vi "AnalysisTools.vi"(7 "Cali.Ref(Caller)":refnum<vi>) -> ()   [LabVIEW 2013]
uses:
  ProcessMethods/Binning/BinType.ctl
  <vilib>/Utility/miscctls.llb/LVRowAndColumnUnsignedTypeDef.ctl
  Files/Signal_Segment.ctl
  ControlDef/ProcessingMode.ctl
  <vilib>/Analysis/6fits.llb/General Linear Fit Algorithm.ctl
  <vilib>/Analysis/6fits.llb/Curve Fitting Criteria.ctl
  UI/Autoscale_Y_Multiple.vi
  ProcessMethods/Binning/SpectraBinning.vi
  ProcessMethods/MassResolutionCalc/FindMassResolution_Multiple.vi
  <vilib>/regexp/Match Regular Expression.xnode
  <vilib>/Analysis/NI_AALPro.lvlib
  <vilib>/Analysis/NI_AAL_SigProc.lvlib
  <vilib>/ptbypt/NI_PtbyPt.lvlib
panel:
  in  "Resolution":bool
  in  "Binning":bool
  in  "BinType":T1
  in  "BinWidth":dbl=1.0 min=0.001 max=32768.0 step=0.001 format="%.3f"
  in  "X++":bool
  in  "X--":bool
  in  "Fullscale X":bool
  in  "Fullscale Y":bool
  in  "Y--":bool
  in  "Y++":bool
  in  "Reload":bool
  in  "Path":path
  out "Spectrum":cluster{dbl[], "Amplitudes":dbl[]}[](graph)
  in  "Calc Calibration":bool
  in  "m/z":dbl
  in  "time":dbl
  in  "Add to":bool
  out "Original m/z":dbl
  in  "Tab Control":T2(tab)
  in  "Calibration Table":dbl[][](array[numeric]) caption="raw m/z"
  in  "Quit":bool
  in  "Export_GraphData":bool
  in  "ApplyToFile":bool
  out "M/z curve fitting":cluster{"Y":dbl[], "Y":dbl[]}[](graph)
  in  "Calibration Coefficients":dbl[](array[numeric]) format="%.5f"
  out "R^2":dbl
  in  "Apply":bool
  in  "mzML Export":bool
  in  "ApplyToMainProgram":bool
  in  "AddSelection":bool
  in  "ExportPCA":bool
  in  "Multicolumn Listbox":i32[](listbox)
  in  "Search":bool
  in  "threshold":dbl format="%#_5p"
  in  "width":i32=3 min=3
  out "# found":i32
  in  "LoadMultiple...":bool
  in  "Reset":bool
  in  "ExportTable":bool
  in  "CopyPeakAreas":bool
  in  "CalcPeakAreas":bool
  in  "Selected Peak list":i32[](listbox)=[2]
  in  "Decode_regexp":string="Br2-Tyr_([-+]?[0-9]*[,\\.]?[0-9]+([eE][-+]?[0-9]+)?)%_([-+]?[0-9]*[,\\.]?[0-9]+([eE][-+]?[0-9]+)?)uJ_([-+]?[0-9]*[,\\.]?[0-9]+([eE][-+]?[0-9]+)?)us_([-+]?[0-9]*[,\\.]?[0-9]+([eE][-+]?[0-9]+)?).txt"
  in  "Decode_Filename?":bool
  in  "Accumulate":bool
  out "Accumulated Data":dbl[][](array[numeric])
  in  "Export+Proc":bool
  out "selected submatch":string
  in  "Submatch Selector":i32
  out "Referance Mass":string[][](table)=[["Compound", "", "mass", ""], ["Sexithiophone", "6T", "493.98", "s"], ["", "4T", "330.00", "s"], ["", "8T", "657.96", "w"], ["NPM", "M+", "297", "s"], ["", "", "217", "w"], ["CHCA", "M+", "189.04", "s"], ["DHB", "M+", "154.03", "s"], ["Rifampcin", "", "", ""], ["Tantalum", "", "", ""], ["Cu", "63", "", ""], ["", "65", "", ""], ["Mo", "", "", ""]]
  # "raw m/z"
  # "time"
  # "cali. m/z"
  # "delta m/z"
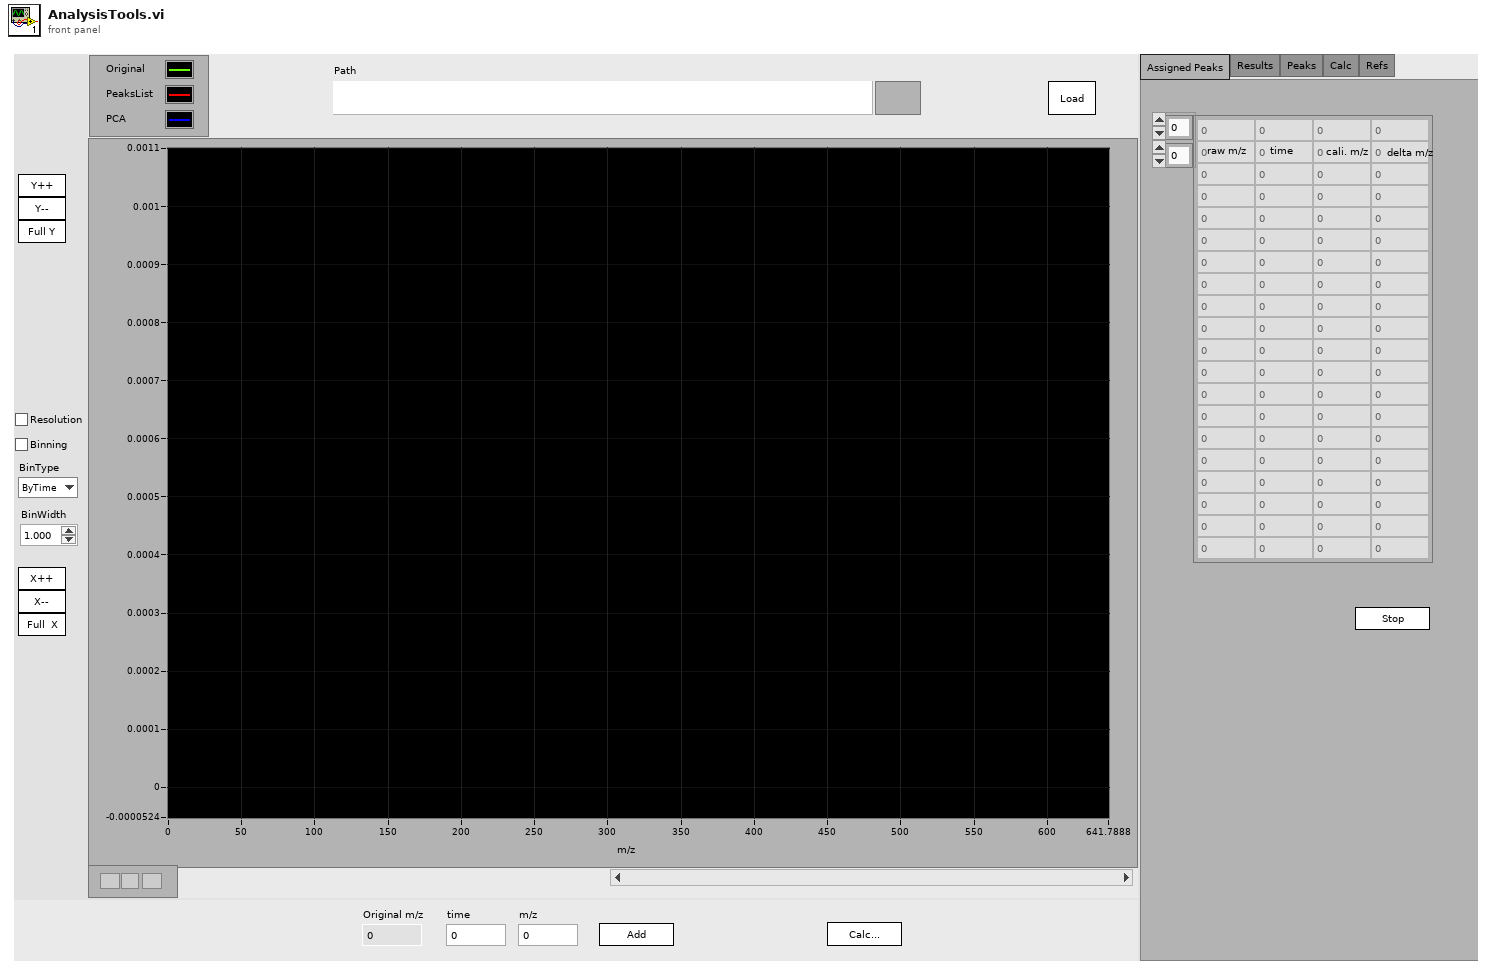
[diagram p1: front panel]
types:
  T1 = typedef "BinType.ctl" = enum16{"ByTime", "ByScreen", "ByMass", "ToUnitMass"}
  T2 = enum32{"Assigned Peaks", "Results", "Peaks", "Calc", "Refs"}
  T3 = typedef "LVRowAndColumnUnsignedTypeDef.ctl" = cluster{"Row":u32, "Column":u32}
  T4 = cluster{"Plot.Bar Plot Style":u8, "Plot.Plot Color":u32, "Plot.Line Style":u8, "Plot.Plot Interpolation":u8, "Plot.Plot Name":string, "Plot.Point Style":u8, "Plot.Visible":bool}[]
  T5 = typedef "Signal_Segment.ctl" = cluster{"SampleRate":dbl, "TrigDelay":dbl, "SpecLength":dbl, "DAQ_Range":dbl, "Average#":i32, "Position":dbl[], "Spectrum":sgl[], "Calibr.":dbl[], "Pressure":dbl, "Desp_LaserEnergy":dbl, "PI_LaserEnergy":dbl, "Voltages Table":sgl[][], "ProcMode":T6, "Threshold":dbl, "Comment":string, "TickCount":dbl, "Time Stamp":timestamp}
  T6 = typedef "ProcessingMode.ctl" = enum16{"None", "Drop by Threshold", "TDC Simulate", "SetFilter"}
  T7 = cluster{"Spectrum":T5, "Peaks Table":dbl[][], "BinnedSpec":cluster{"m/z":dbl[], "Intensity":dbl[]}, "PeaksList":cluster{"m/z":dbl[], "Intensity":dbl[]}, "PCA":cluster{"m/z":dbl[], "Intensity":dbl[]}, "m/z":dbl[], "InitialCali.":dbl[], "Filename":string, "AccumulatedPeakAreas":cluster{"Labels":string[], "Areas":dbl[][], "Areas^2":dbl[][], "n":i32[]}, "app vi reference":refnum<vi>}
  T8 = cluster{"Labels":string[], "Areas":dbl[][], "Areas^2":dbl[][], "n":i32[]}
  T9 = typedef "LVPoint32TypeDef.ctl" = cluster{"Horizontal":i32, "Vertical":i32}
  T10 = typedef "NI_AALPro.lvlib/Curve Fitting Criteria.ctl" = u16
  T11 = typedef "NI_AALPro.lvlib/General Linear Fit Algorithm.ctl" = u16
  T12 = cluster{"Calibration Table":dbl[], "Calibration Table":dbl[]}
  T13 = cluster{"Calibration Table":dbl[], "Calibration Table":dbl[]}[]
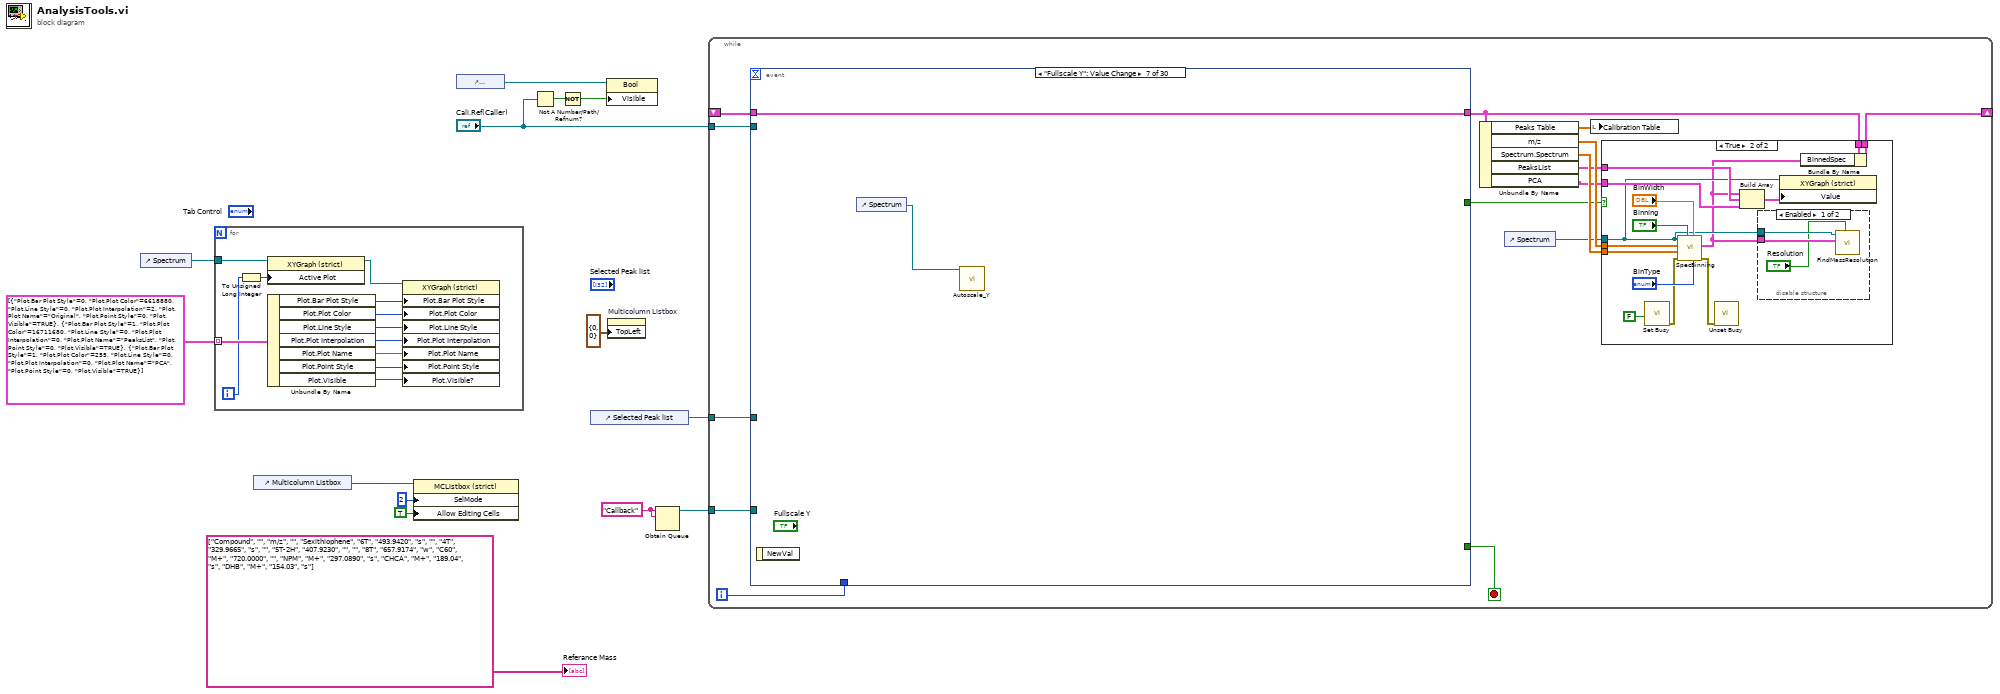
[diagram p0: block diagram]
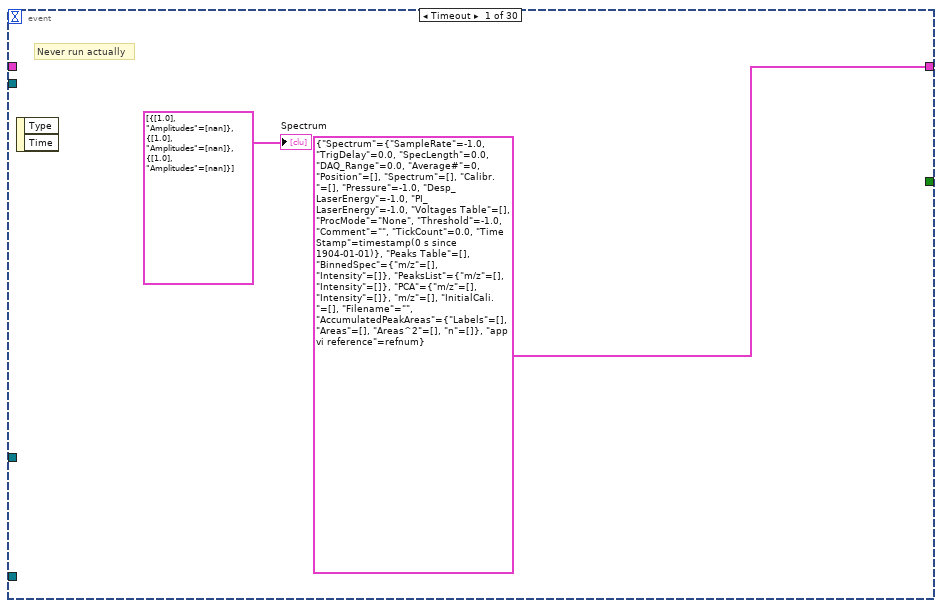
[diagram p4: hidden frame]
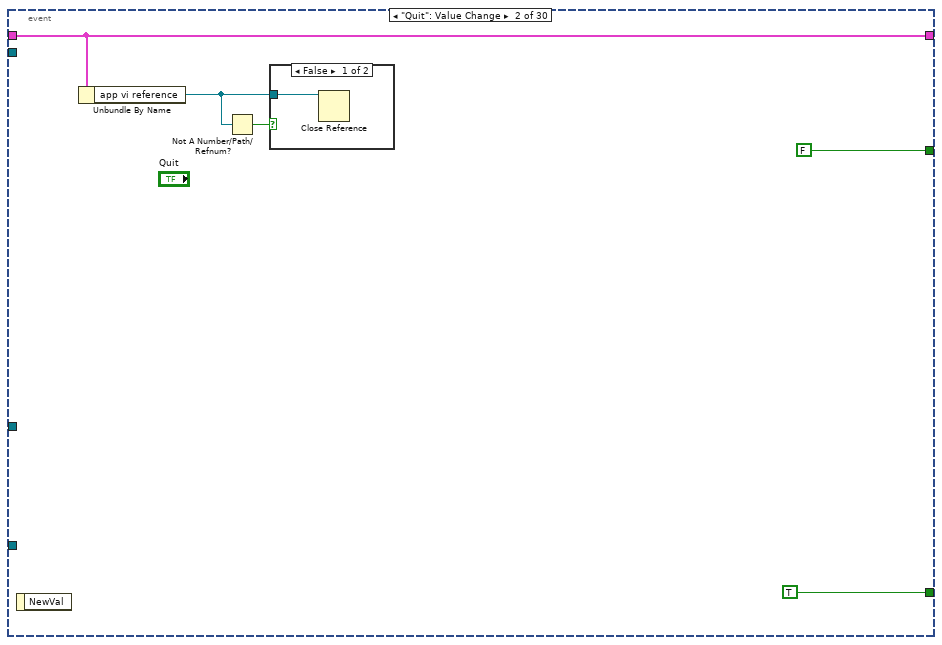
[diagram p5: hidden frame]
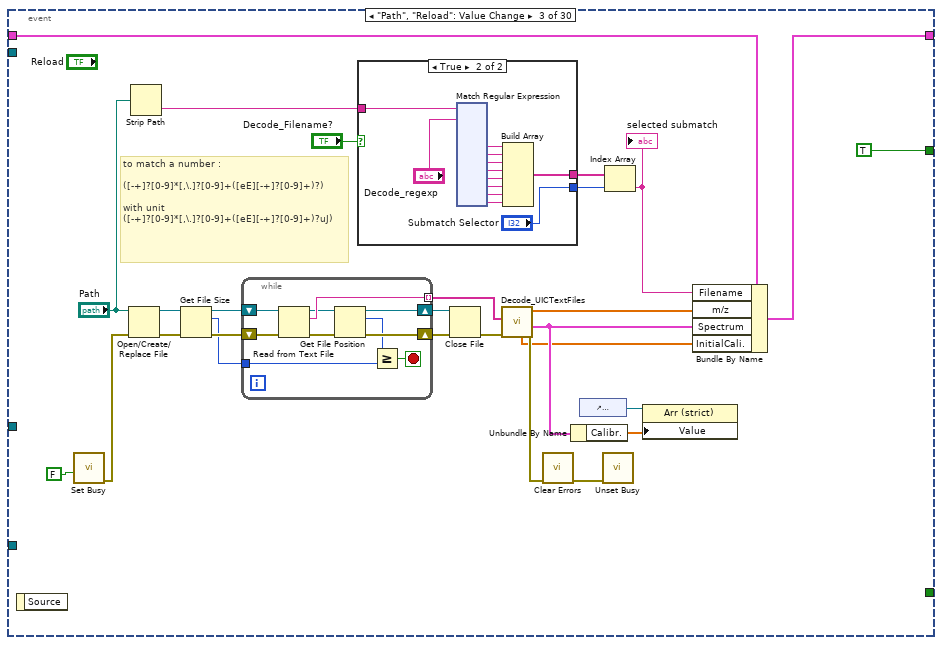
[diagram p7: hidden frame]
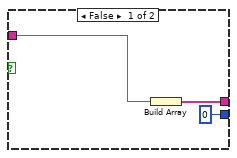
[diagram p8: hidden frame]
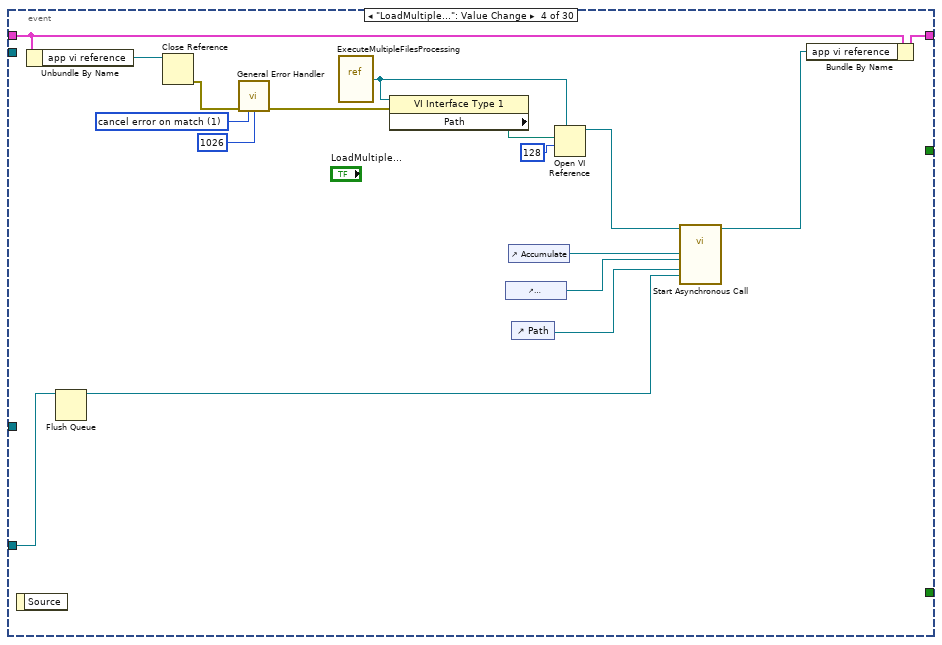
[diagram p9: hidden frame]
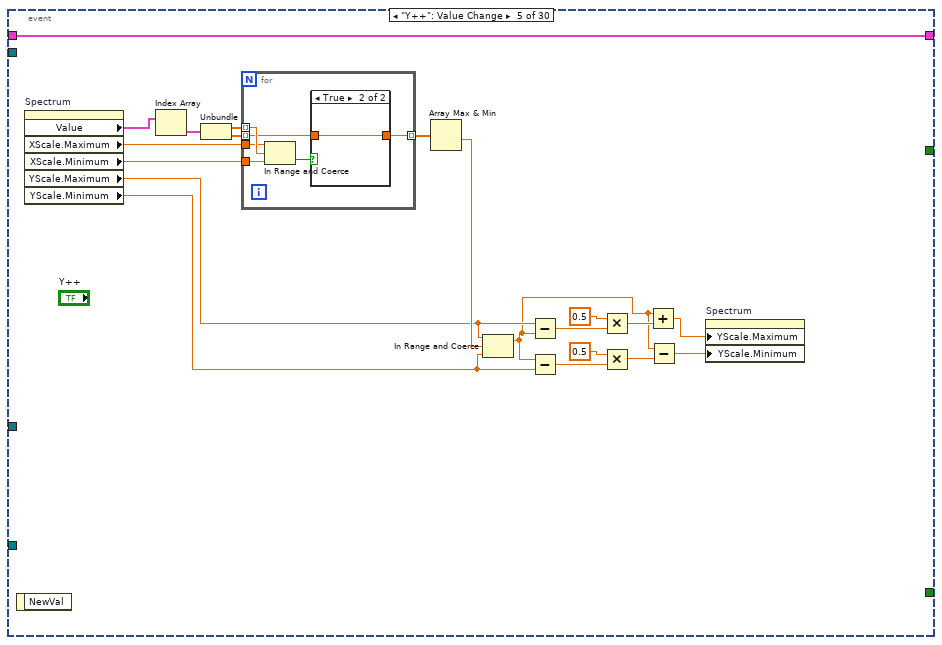
[diagram p10: hidden frame]
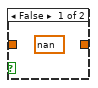
[diagram p11: hidden frame]
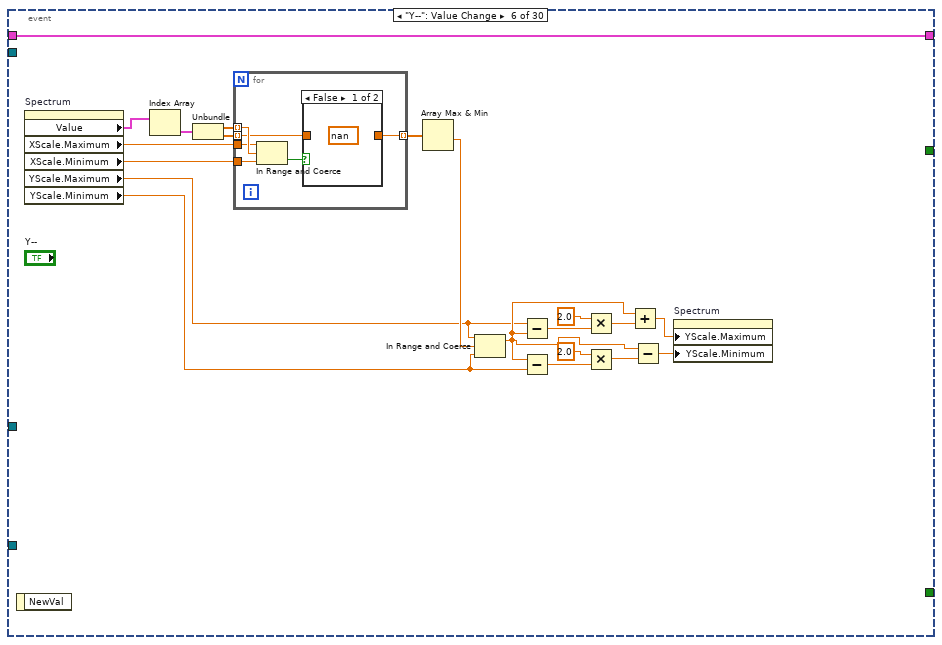
[diagram p12: hidden frame]
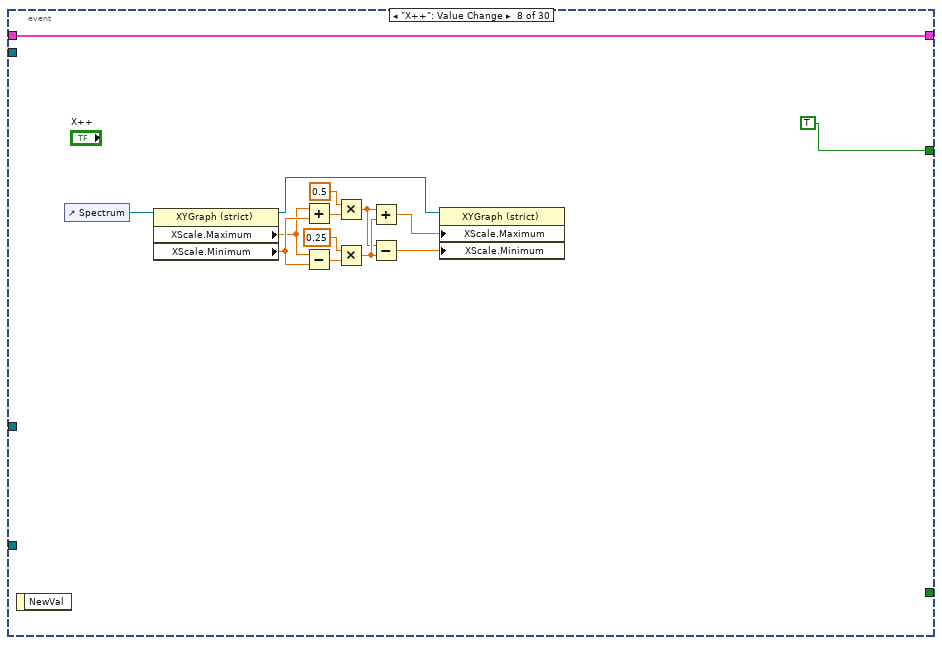
[diagram p14: hidden frame]
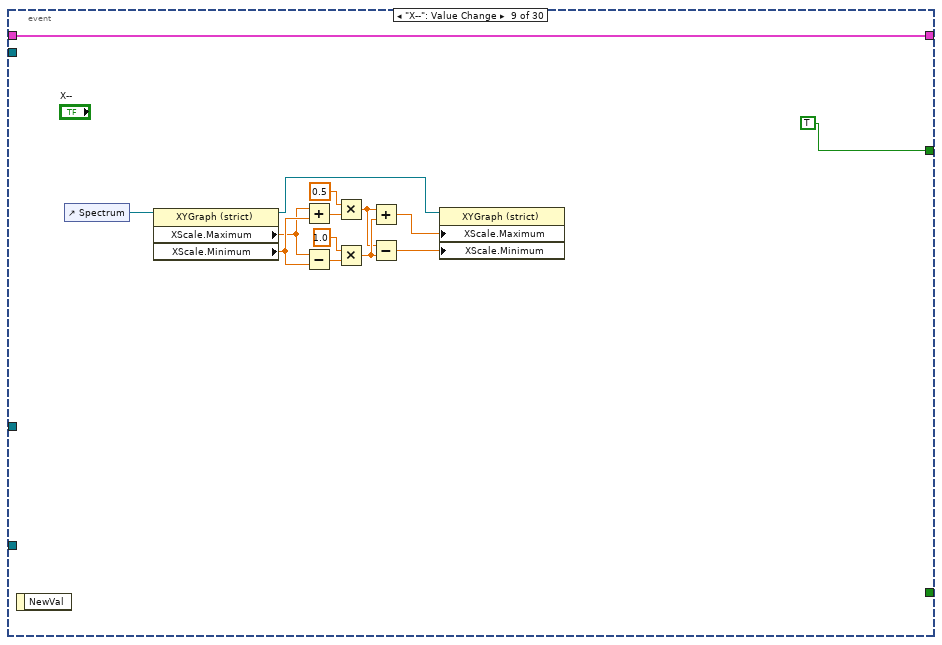
[diagram p15: hidden frame]
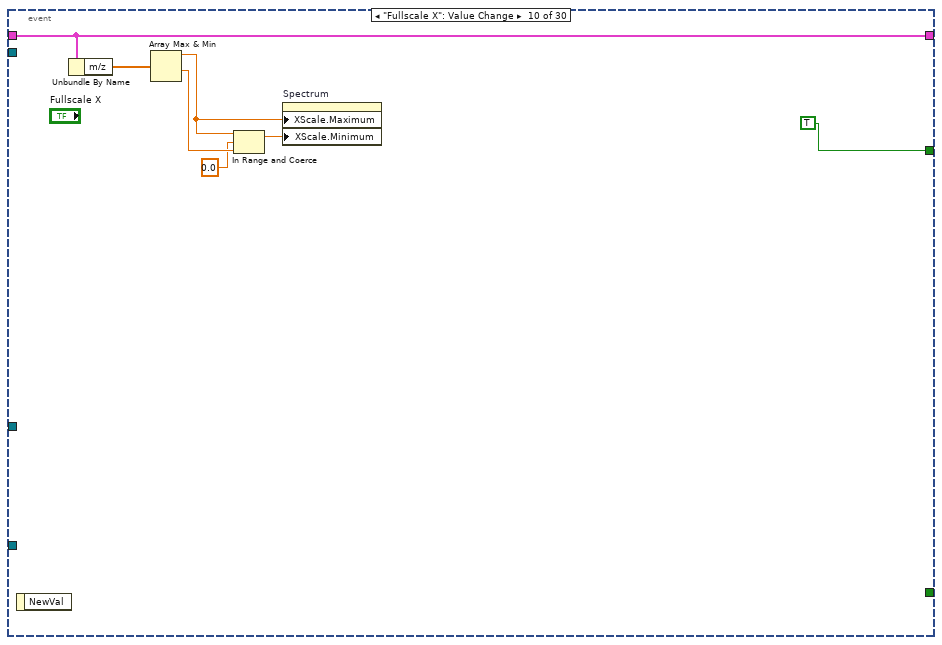
[diagram p16: hidden frame]
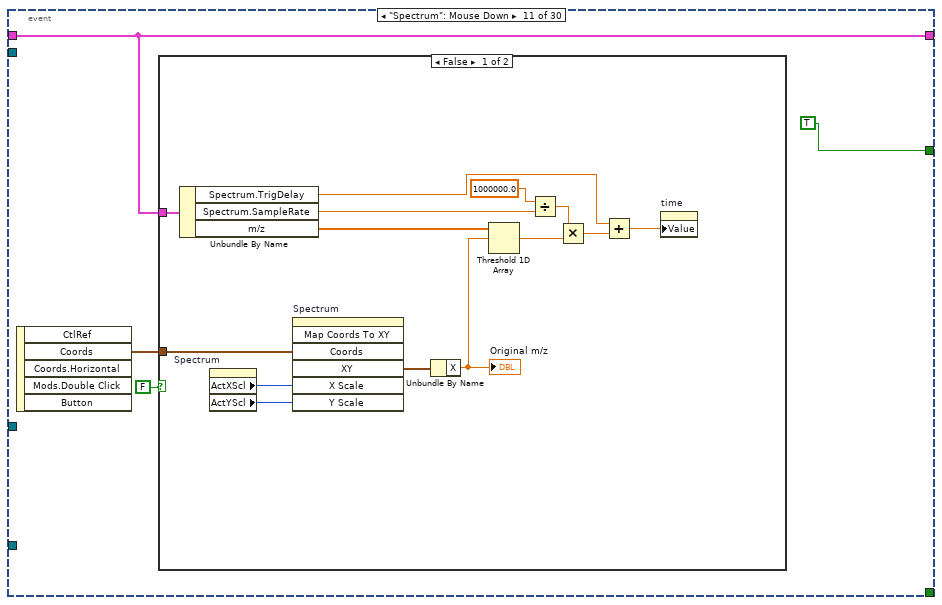
[diagram p17: hidden frame]
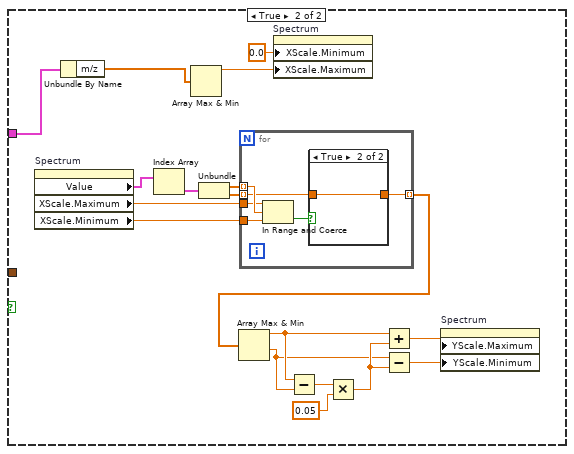
[diagram p18: hidden frame]
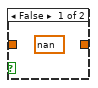
[diagram p19: hidden frame]
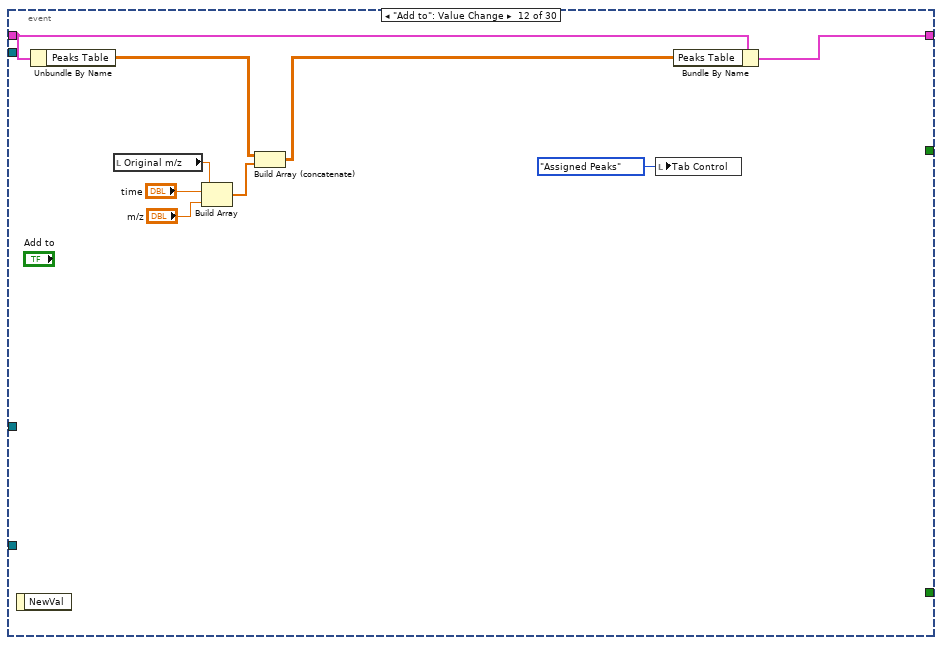
[diagram p20: hidden frame]
diagram:
  w7 = "Callback" ("name (unnamed)")
  n1 = control-ref of="Spectrum"() -> (w12:refnum<vi>)
  n2 = for {
    tunnel: w12 -> [w26]
    tunnel: T4 [{"Plot.Bar Plot Style"=0, "Plot.Plot Color"=6618880, "Plot.Line Style"=0, "Plot.Plot Interpolation"=2, "Plot.Plot Name"="Original", "Plot.Point Style"=0, "Plot.Visible"=TRUE}, {"Plot.Bar Plot Style"=1, "Plot.Plot Color"=16711680, "Plot.Line Style"=0, "Plot.Plot Interpolation"=0, "Plot.Plot Name"="PeaksList", "Plot.Point Style"=0, "Plot.Visible"=TRUE}, {"Plot.Bar Plot Style"=1, "Plot.Plot Color"=255, "Plot.Line Style"=0, "Plot.Plot Interpolation"=0, "Plot.Plot Name"="PCA", "Plot.Point Style"=0, "Plot.Visible"=TRUE}] -> [w24] mode=indexing
    i -> [w16]
    n3 = To Unsigned Long Integer(number=w16) -> (unsigned 32bit integer=w15:u32)
    n4 = property class="XYGraph (strict)"(reference=w26, "Active Plot"=w15) -> (reference out=w25:refnum<vi>)  [unwired: 1 in, 1 out]
    n5 = Unbundle By Name(w24) -> ("Plot.Bar Plot Style"=w19:u8, "Plot.Plot Color"=w20:u32, "Plot.Line Style"=w17:u8, "Plot.Plot Interpolation"=w18:u8, "Plot.Plot Name"=w21:string, "Plot.Point Style"=w22:u8, "Plot.Visible"=w23:bool)
    n6 = property class="XYGraph (strict)"(reference=w25, "Plot.Bar Plot Style"=w19, "Plot.Plot Color"=w20, "Plot.Line Style"=w17, "Plot.Plot Interpolation"=w18, "Plot.Plot Name"=w21, "Plot.Point Style"=w22, "Plot.Visible?"=w23) -> ()  [unwired: 1 in, 2 out]
  }
  n7 = control-ref of="Multicolumn Listbox"() -> (w11:refnum<vi>)
  n8 = property class="MCListbox (strict)"(reference=w11, "SelMode"=2 ("Selection Mode"), "Allow Editing Cells"=TRUE) -> ()  [unwired: 1 in, 2 out]
  n9 = control-ref of="ApplyToMainProgram"() -> (w2:refnum<vi>)
  n10 = Not A Number/Path/Refnum?(number/path/refnum="Cali.Ref(Caller)") -> (NaN/Path/Refnum?=w4:bool)
  n11 = Not(x=w4) -> (.not. x?=w3:bool)
  n12 = control-ref of="Selected Peak list"() -> (w5:refnum<vi>)
  n13 = property class="Bool"(reference=w2, "Visible"=w3) -> ()  [unwired: 1 in, 2 out]
  n14 = property on="Multicolumn Listbox" class="MCListbox (strict)"("TopLeft"=T3 {"Row"=0, "Column"=0} ("Top Left Visible Cell")) -> ()  [unwired: 2 in, 2 out]
  n15 = Obtain Queue(name (unnamed)=w7, element data type=w7) -> (queue out=w6:refnum<queue>)  [unwired: 3 in, 2 out]
  n16 = while {
    shift-right: [w34] -> _
    shift-left: _ -> [w41]
    tunnel: w6 -> [w29]
    tunnel: w5 -> [w28]
    tunnel: "Cali.Ref(Caller)" -> [w27]
    i -> [w30]
    stop <- w39 stop-if-true
    n17 = event shown="[6] \"Fullscale Y\": Value Change" {
      selector: _ -> [_ _ _ _ _ _ _ _ _ _ _ _ _ _ _ _ _ _ _ _ _ _ _ _ _ _ _ _ _ _]
      dyn-events: _ -> [_ _ _ _ _ _ _ _ _ _ _ _ _ _ _ _ _ _ _ _ _ _ _ _ _ _ _ _ _ _]
      timeout: _ -> [_ _ _ _ _ _ _ _ _ _ _ _ _ _ _ _ _ _ _ _ _ _ _ _ _ _ _ _ _ _]
      tunnel: [T7 {"Spectrum"={"SampleRate"=-1.0, "TrigDelay"=0.0, "SpecLength"=0.0, "DAQ_Range"=0.0, "Average#"=0, "Position"=[], "Spectrum"=[], "Calibr."=[], "Pressure"=-1.0, "Desp_LaserEnergy"=-1.0, "PI_LaserEnergy"=-1.0, "Voltages Table"=[], "ProcMode"=enum."None", "Threshold"=-1.0, "Comment"="", "TickCount"=0.0, "Time Stamp"=timestamp(0 s since 1904-01-01)}, "Peaks Table"=[], "BinnedSpec"={"m/z"=[], "Intensity"=[]}, "PeaksList"={"m/z"=[], "Intensity"=[]}, "PCA"={"m/z"=[], "Intensity"=[]}, "m/z"=[], "InitialCali."=[], "Filename"="", "AccumulatedPeakAreas"={"Labels"=[], "Areas"=[], "Areas^2"=[], "n"=[]}, "app vi reference"=refnum} w65 w95 w251 w277 w304 w316 w330 w344 w351 w354 w401 w405 w446 w481 w501 w532 w535 w545 w663 w693 w736 w740 w745 w870 w891 w913 w931 w964 w1005] -> w35
      tunnel: w41 -> [_ w65 w94 w249 w277 w304 w316 w330 w344 w351 w354 w402 w405 w438 w480 w501 w532 w535 w545 w664 w694 w736 w741 w745 w870 w891 w913 w931 w965 w1006]
      tunnel: [_ TRUE _ _ _ _ _ _ _ _ _ _ _ _ _ _ _ _ _ _ _ _ _ _ _ _ _ _ _ _] -> w39
      tunnel: [_ FALSE TRUE _ _ _ _ TRUE TRUE TRUE TRUE _ TRUE TRUE TRUE TRUE _ _ _ TRUE _ _ _ _ _ _ _ _ _ _] -> w36
      tunnel: w30 -> [_ _ _ _ _ _ _ _ _ _ _ _ _ _ _ _ _ _ _ _ _ _ _ _ _ _ _ _ _ _]
      tunnel: w29 -> [_ _ _ w253 _ _ _ _ _ _ _ _ _ _ _ _ _ _ _ _ _ _ _ _ _ _ _ _ w962 _]
      tunnel: w28 -> [_ _ _ _ _ _ _ _ _ _ _ _ _ _ _ _ _ _ _ _ _ _ _ _ _ _ _ _ w961 _]
      tunnel: w27 -> [_ _ _ _ _ _ _ _ _ _ _ _ _ _ _ _ _ w533 _ _ _ _ _ _ _ _ _ _ _ _]
      event Timeout {
        # "Never run actually"
        n18 = event-data() -> ()  [unwired: 1 in, 2 out]
        "Spectrum" <- cluster{dbl[], "Amplitudes":dbl[]}[] [{[1.0], "Amplitudes"=[nan]}, {[1.0], "Amplitudes"=[nan]}, {[1.0], "Amplitudes"=[nan]}]
      }
      event "Quit": Value Change {
        n19 = event-data() -> ()  [unwired: 1 in, 1 out]
        n20 = Unbundle By Name(w65) -> ("app vi reference"=w63:refnum<vi>)
        n21 = Not A Number/Path/Refnum?(number/path/refnum=w63) -> (NaN/Path/Refnum?=w64:bool)
        n22 = case shown="False" w64 {
          tunnel: w63 -> [w68 _]
          frame False {
            n23 = Close Reference(reference=w68) -> ()  [unwired: 1 in, 1 out]
          }
          frame True {
          }
        }
      }
      event "Path", "Reload": Value Change {
        # "to match a number :\n\n([-+]?[0-9]*[,\\.]?[0-9]+([eE][-+]?[0-9]+)?)\n\nwith unit \n([-+]?[0-9]*[,\\.]?[0-9]+([eE][-+]?[0-9]+)?uJ)"
        n24 = event-data() -> ()  [unwired: 1 in, 1 out]
        n25 = call <vilib>:"Set Busy.vi"("disable click? (T)"=FALSE) -> ("error out"=w84:errorcluster)  [unwired: 9 in, 1 out]
        n26 = Open/Create/Replace File(file path (use dialog)="Path", error in=w84) -> (refnum out=w92:refnum<file>, error out=w93:errorcluster)  [unwired: 4 in, 1 out]
        n27 = Strip Path(path="Path") -> (name=w73:string)  [unwired: 1 out]
        n28 = Get File Size(file=w92, error in=w93) -> (refnum out=w90:refnum<file>, size (in bytes)=w88:i64, 0:w91:errorcluster)
        n29 = while {
          shift-right: [w239] -> w78
          shift-left: w90 -> [w243]
          shift-right: [w238] -> w77
          shift-left: w91 -> [w242]
          tunnel: [w241] -> w89 mode=indexing
          tunnel: w88 -> [w235]
          stop <- w234 stop-if-true
          n30 = Read from Text File(file (use dialog)=w243, error in=w242) -> (refnum out=w240:refnum<file>, text=w241:string, error out=w237:errorcluster)  [unwired: 2 in, 1 out]
          n31 = Get File Position(4:w237, 7:w240) -> (0:w238:errorcluster, 2:w236:i64, 3:w239:refnum<file>)
          n32 = Greater Or Equal?(x=w236, y=w235) -> (x >= y?=w234:bool)
        }
        n33 = case shown="True" "Decode_Filename?" {
          tunnel: w73 -> [w97 w109]
          tunnel: [w98 w100] -> w70
          tunnel: [0 ("Submatch Selector") "Submatch Selector"] -> w69
          frame False {
            n34 = Build Array(w97) -> (w98:string[])
          }
          frame True {
            n35 = xnode "Match Regular Expression"("input string"=w109, "regular expression"="Decode_regexp") -> ("submatch 1"=w108:string, "submatch 2"=w107:string, "submatch 3"=w106:string, "submatch 4"=w105:string, "submatch 5"=w104:string, "submatch 6"=w103:string, "submatch 7"=w102:string, "submatch 8"=w101:string)  [unwired: 4 in, 5 out]
            n36 = Build Array(w108, w107, w106, w105, w104, w103, w102, w101) -> (w100:string[])
          }
        }
        n37 = Close File(refnum=w78, error in=w77) -> (error out=w76:errorcluster)  [unwired: 1 out]
        n38 = call "Decode_UICTextFiles.vi"("error in"=w76, "Text Array"=w89) -> ("error out"=w87:errorcluster, "Spectrum"=w81:T5, "m/z list"=w82:dbl[], "InitialCali."=w75:dbl[])  [unwired: 5 in, 1 out]
        n39 = call <vilib>:"Clear Errors.vi"("error in (no error)"=w87) -> ("error out"=w83:errorcluster)  [unwired: 6 in]
        n40 = Unbundle By Name(w81) -> ("Calibr."=w79:dbl[])
        n41 = control-ref of="Calibration Coefficients"() -> (w80:refnum<vi>)
        n42 = call <vilib>:"Unset Busy.vi"("error in (no error)"=w83) -> ()  [unwired: 10 in, 1 out]
        n43 = Index Array(array=w70, index=w69) -> (element=w71:string)
        "selected submatch" <- w71
        n44 = property class="Arr (strict)"(reference=w80, "Value"=w79) -> ()  [unwired: 1 in, 2 out]
        n45 = Bundle By Name(cluster=w94, "Filename"=w71, "m/z"=w82, "Spectrum"=w81, "InitialCali."=w75) -> (w95:T7)
      }
      event "LoadMultiple...": Value Change {
        w245 = 1 items=["no exception", "cancel error on match", "set error on match"] ("[exception action] (none:0)")
        n46 = event-data() -> ()  [unwired: 1 in, 1 out]
        n47 = Unbundle By Name(w249) -> ("app vi reference"=w248:refnum<vi>)
        n48 = Flush Queue(queue=w253) -> (queue out=w252:refnum<queue>)  [unwired: 1 in, 2 out]
        n49 = Close Reference(reference=w248) -> (error out=w247:errorcluster)  [unwired: 1 in]
        n50 = call <vilib>:"General Error Handler.vi"("error in (no error)"=w247, "[exception action] (none:0)"=w245, "[exception code]"=1026) -> ("error out"=w246:errorcluster)  [unwired: 8 in, 4 out]
        n51 = vi-ref "ExecuteMultipleFilesProcessing.vi"() -> (w260:refnum<vi>)
        n52 = property class="VI Interface Type 1"(reference=w260, error in=w246) -> ("Path"=w259:path)  [unwired: 2 out]
        n53 = control-ref of="CalcPeakAreas"() -> (w255:refnum<vi>)
        n54 = control-ref of="Accumulate"() -> (w256:refnum<vi>)
        n55 = control-ref of="Path"() -> (w254:refnum<vi>)
        n56 = Open VI Reference(type specifier VI Refnum (for type only)=w260, vi path=w259, options=128) -> (vi reference=w257:refnum<vi>)  [unwired: 3 in, 1 out]
        n57 = call-by-ref "Start Asynchronous Call"(reference=w257, "Callback queue in"=w252, "Path"=w254, "CalcPeakAreas"=w255, "Accumulate"=w256) -> (reference out=w250:refnum<vi>)  [unwired: 9 in, 1 out]
        n58 = Bundle By Name(cluster=w249, "app vi reference"=w250) -> (w251:T7)
      }
      event "Y++": Value Change {
        n59 = event-data() -> ()  [unwired: 1 in, 1 out]
        n60 = property on="Spectrum" class="XYGraph (strict)"() -> ("Value"=w266:cluster{dbl[], "Amplitudes":dbl[]}[], "XScale.Maximum"=w274:dbl, "XScale.Minimum"=w273:dbl, "YScale.Maximum"=w263:dbl, "YScale.Minimum"=w262:dbl)  [unwired: 2 in, 2 out]
        n61 = Index Array(array=w266) -> (element=w265:cluster{dbl[], "Amplitudes":dbl[]})  [unwired: 1 in]
        n62 = Unbundle(w265) -> (w276:dbl[], "Amplitudes"=w275:dbl[])
        n63 = for {
          tunnel: w275 -> [w282] mode=indexing
          tunnel: w276 -> [w286] mode=indexing
          tunnel: w273 -> [w285]
          tunnel: w274 -> [w284]
          tunnel: [w281] -> w272 mode=indexing
          n64 = In Range and Coerce(upper limit=w284, x=w286, lower limit=w285) -> (In Range?=w283:bool)  [unwired: 1 out]
          n65 = case shown="True" w283 {
            tunnel: w282 -> [_ w287]
            tunnel: [_ w287] -> w281
            frame False {
              (unwired) nan
            }
            frame True {
            }
          }
        }
        n66 = Array Max & Min(array=w272) -> (min value=w264:dbl)  [unwired: 3 out]
        n67 = In Range and Coerce(upper limit=w263, x=w264, lower limit=w262) -> (coerced(x)=w261:dbl)  [unwired: 1 out]
        n68 = Subtract(x=w263, y=w261) -> (x-y=w271:dbl)
        n69 = Subtract(x=w261, y=w262) -> (x-y=w269:dbl)
        n70 = Multiply(x=0.5, y=w271) -> (x*y=w279:dbl)
        n71 = Multiply(x=0.5, y=w269) -> (x*y=w268:dbl)
        n72 = Add(x=w261, y=w279) -> (x+y=w278:dbl)
        n73 = Subtract(x=w261, y=w268) -> (x-y=w267:dbl)
        n74 = property on="Spectrum" class="XYGraph (strict)"("YScale.Maximum"=w278, "YScale.Minimum"=w267) -> ()  [unwired: 2 in, 2 out]
      }
      event "Y--": Value Change {
        n75 = event-data() -> ()  [unwired: 1 in, 1 out]
        n76 = property on="Spectrum" class="XYGraph (strict)"() -> ("Value"=w303:cluster{dbl[], "Amplitudes":dbl[]}[], "XScale.Maximum"=w300:dbl, "XScale.Minimum"=w299:dbl, "YScale.Maximum"=w289:dbl, "YScale.Minimum"=w288:dbl)  [unwired: 2 in, 2 out]
        n77 = Index Array(array=w303) -> (element=w292:cluster{dbl[], "Amplitudes":dbl[]})  [unwired: 1 in]
        n78 = Unbundle(w292) -> (w302:dbl[], "Amplitudes"=w301:dbl[])
        n79 = for {
          tunnel: w301 -> [w309] mode=indexing
          tunnel: w302 -> [w313] mode=indexing
          tunnel: w299 -> [w312]
          tunnel: w300 -> [w311]
          tunnel: [w308] -> w298 mode=indexing
          n80 = In Range and Coerce(upper limit=w311, x=w313, lower limit=w312) -> (In Range?=w310:bool)  [unwired: 1 out]
          n81 = case shown="False" w310 {
            tunnel: w309 -> [_ w314]
            tunnel: [_ w314] -> w308
            frame False {
              (unwired) nan
            }
            frame True {
            }
          }
        }
        n82 = Array Max & Min(array=w298) -> (min value=w290:dbl)  [unwired: 3 out]
        n83 = In Range and Coerce(upper limit=w289, x=w290, lower limit=w288) -> (coerced(x)=w291:dbl)  [unwired: 1 out]
        n84 = Subtract(x=w289, y=w291) -> (x-y=w297:dbl)
        n85 = Subtract(x=w291, y=w288) -> (x-y=w295:dbl)
        n86 = Multiply(x=2.0, y=w297) -> (x*y=w306:dbl)
        n87 = Multiply(x=2.0, y=w295) -> (x*y=w294:dbl)
        n88 = Add(x=w291, y=w306) -> (x+y=w305:dbl)
        n89 = Subtract(x=w291, y=w294) -> (x-y=w293:dbl)
        n90 = property on="Spectrum" class="XYGraph (strict)"("YScale.Maximum"=w305, "YScale.Minimum"=w293) -> ()  [unwired: 2 in, 2 out]
      }
      event "Fullscale Y": Value Change {
        n91 = event-data() -> ()  [unwired: 1 in, 1 out]
        n92 = control-ref of="Spectrum"() -> (w315:refnum<vi>)
        n93 = call-poly "Autoscale_Y.vi"("GraphRef"=w315) -> ()  [unwired: 11 in]
      }
      event "X++": Value Change {
        n94 = event-data() -> ()  [unwired: 1 in, 1 out]
        n95 = control-ref of="Spectrum"() -> (w319:refnum<vi>)
        n96 = property on="Property Node" class="XYGraph (strict)"(reference=w319) -> (reference out=w318:refnum<vi>, "XScale.Maximum"=w320:dbl, "XScale.Minimum"=w321:dbl)  [unwired: 1 in, 1 out]
        n97 = Add(x=w320, y=w321) -> (x+y=w322:dbl)
        n98 = Subtract(x=w320, y=w321) -> (x-y=w325:dbl)
        n99 = Multiply(x=0.5, y=w322) -> (x*y=w326:dbl)
        n100 = Multiply(x=0.25, y=w325) -> (x*y=w327:dbl)
        n101 = Add(x=w326, y=w327) -> (x+y=w328:dbl)
        n102 = Subtract(x=w326, y=w327) -> (x-y=w329:dbl)
        n103 = property on="Property Node" class="XYGraph (strict)"(reference=w318, "XScale.Maximum"=w328, "XScale.Minimum"=w329) -> ()  [unwired: 1 in, 2 out]
      }
      event "X--": Value Change {
        n104 = event-data() -> ()  [unwired: 1 in, 1 out]
        n105 = control-ref of="Spectrum"() -> (w333:refnum<vi>)
        n106 = property on="Property Node" class="XYGraph (strict)"(reference=w333) -> (reference out=w332:refnum<vi>, "XScale.Maximum"=w334:dbl, "XScale.Minimum"=w335:dbl)  [unwired: 1 in, 1 out]
        n107 = Add(x=w334, y=w335) -> (x+y=w336:dbl)
        n108 = Subtract(x=w334, y=w335) -> (x-y=w339:dbl)
        n109 = Multiply(x=0.5, y=w336) -> (x*y=w340:dbl)
        n110 = Multiply(x=1.0, y=w339) -> (x*y=w341:dbl)
        n111 = Add(x=w340, y=w341) -> (x+y=w342:dbl)
        n112 = Subtract(x=w340, y=w341) -> (x-y=w343:dbl)
        n113 = property on="Property Node" class="XYGraph (strict)"(reference=w332, "XScale.Maximum"=w342, "XScale.Minimum"=w343) -> ()  [unwired: 1 in, 2 out]
      }
      event "Fullscale X": Value Change {
        n114 = event-data() -> ()  [unwired: 1 in, 1 out]
        n115 = Unbundle By Name(w351) -> ("m/z"=w345:dbl[])
        n116 = Array Max & Min(array=w345) -> (max value=w346:dbl, min value=w349:dbl)  [unwired: 2 out]
        n117 = In Range and Coerce(upper limit=w346, x=0.0 ("X Scale.Range:Minimum"), lower limit=w349) -> (coerced(x)=w347:dbl)  [unwired: 1 out]
        n118 = property on="Spectrum" class="XYGraph (strict)"("XScale.Maximum"=w346, "XScale.Minimum"=w347) -> ()  [unwired: 2 in, 2 out]
      }
      event "Spectrum": Mouse Down {
        n119 = event-data() -> ("Coords"=w355:T9)  [unwired: 1 in, 4 out]
        n120 = case shown="False" FALSE {
          tunnel: w355 -> [w369 _]
          tunnel: w354 -> [w365 w385]
          frame False {
            n121 = Unbundle By Name(w365) -> ("Spectrum.TrigDelay"=w357:dbl, "Spectrum.SampleRate"=w356:dbl, "m/z"=w359:dbl[])
            n122 = property on="Spectrum" class="XYGraph (strict)"() -> ("ActXScl"=w368:i32, "ActYScl"=w367:i32)  [unwired: 2 in, 2 out]
            n123 = invoke on="Spectrum" class="XYGraph (strict)" method="Map Coords To XY"("Coords"=w369, "X Scale"=w368, "Y Scale"=w367) -> ("XY"=w366:cluster{"X":dbl, "Y":dbl})  [unwired: 4 in, 6 out]
            n124 = Unbundle By Name(w366) -> ("X"=w360:dbl)
            "Original m/z" <- w360
            n125 = Threshold 1D Array(2:w360, 3:w359) -> (0:w362:dbl)  [unwired: 1 in]
            n126 = Divide(x=1000000.0, y=w356) -> (x/y=w363:dbl)
            n127 = Multiply(x=w363, y=w362) -> (x*y=w361:dbl)
            n128 = Add(x=w357, y=w361) -> (x+y=w358:dbl)
            n129 = property on="time" class="DigNum (strict)"("Value"=w358) -> ()  [unwired: 2 in, 2 out]
          }
          frame True {
            n130 = property on="Spectrum" class="XYGraph (strict)"() -> ("Value"=w384:cluster{dbl[], "Amplitudes":dbl[]}[], "XScale.Maximum"=w381:dbl, "XScale.Minimum"=w380:dbl)  [unwired: 2 in, 2 out]
            n131 = Unbundle By Name(w385) -> ("m/z"=w370:dbl[])
            n132 = Index Array(array=w384) -> (element=w371:cluster{dbl[], "Amplitudes":dbl[]})  [unwired: 1 in]
            n133 = Array Max & Min(array=w370) -> (max value=w386:dbl)  [unwired: 3 out]
            n134 = Unbundle(w371) -> (w383:dbl[], "Amplitudes"=w382:dbl[])
            n135 = for {
              tunnel: w382 -> [w389] mode=indexing
              tunnel: w383 -> [w393] mode=indexing
              tunnel: w380 -> [w392]
              tunnel: w381 -> [w391]
              tunnel: [w388] -> w372 mode=indexing
              n136 = In Range and Coerce(upper limit=w391, x=w393, lower limit=w392) -> (In Range?=w390:bool)  [unwired: 1 out]
              n137 = case shown="True" w390 {
                tunnel: w389 -> [_ w394]
                tunnel: [_ w394] -> w388
                frame False {
                  (unwired) nan
                }
                frame True {
                }
              }
            }
            n138 = Array Max & Min(array=w372) -> (max value=w374:dbl, min value=w373:dbl)  [unwired: 2 out]
            n139 = property on="Spectrum" class="XYGraph (strict)"("XScale.Minimum"=0.0 ("X Scale.Range:Minimum"), "XScale.Maximum"=w386) -> ()  [unwired: 2 in, 2 out]
            n140 = Subtract(x=w374, y=w373) -> (x-y=w377:dbl)
            n141 = Multiply(x=w377, y=0.05) -> (x*y=w375:dbl)
            n142 = Add(x=w374, y=w375) -> (x+y=w379:dbl)
            n143 = Subtract(x=w373, y=w375) -> (x-y=w378:dbl)
            n144 = property on="Spectrum" class="XYGraph (strict)"("YScale.Maximum"=w379, "YScale.Minimum"=w378) -> ()  [unwired: 2 in, 2 out]
          }
        }
      }
      event "Add to": Value Change {
        n145 = event-data() -> ()  [unwired: 1 in, 1 out]
        n146 = Unbundle By Name(w402) -> ("Peaks Table"=w403:dbl[][])
        n147 = local read "Original m/z"() -> (w398:dbl)
        n148 = Build Array(w398, "time", "m/z") -> (w396:dbl[])
        n149 = Build Array (concatenate)(w403, w396) -> (w397:dbl[][])
        n150 = local write "Tab Control"(T2."Assigned Peaks" ("Tab Control")) -> ()
        n151 = Bundle By Name(cluster=w402, "Peaks Table"=w397) -> (w401:T7)
      }
      event "Spectrum": Scale Range Change; "Binning", "BinWidth", "Resolution": Value Change {
        n152 = event-data() -> ()  [unwired: 1 in, 1 out]
      }
      event "Calc Calibration": Value Change {
        w424 = "\n"
        w452 = 100
        w457 = T10 0 items=["Least Square", "Least Absolute Residual", "Bisquare"] ("method")
        w458 = T11 0 items=["SVD", "Givens", "Givens2", "Householder", "LU Decomposition", "Cholesky", "SVD for Rank Deficient H"] ("algorithm")
        n153 = event-data() -> ()  [unwired: 1 in, 1 out]
        n154 = Unbundle By Name(w438) -> ("BinnedSpec.Intensity"=w437:dbl[], "Spectrum.TrigDelay"=w417:dbl, "Spectrum.SampleRate"=w418:dbl)
        n155 = Index Array(array="Calibration Table", index (col) #1=1 ("disabled index (col)"), index (col) #2=2 ("index (col)")) -> (element #1=w416:dbl[], element #2=w409:dbl[])  [unwired: 2 in]
        n156 = Index Array(array="Calibration Table", index (col)=2 ("disabled index (col)")) -> (element=w432:dbl[])  [unwired: 1 in]
        n157 = Divide(x=1000000.0, y=w418) -> (x/y=w419:dbl)
        n158 = Array Size(array=w437) -> (size(s)=w436:i32)
        n159 = Multiply(x=w417, y=w419) -> (x*y=w420:dbl)
        n160 = call <vilib>:"General Polynomial Fit.vi"("Y"=w409, "polynomial order"=2, "X"=w416, "method"=w457, "algorithm"=w458) -> ("Best Polynomial Fit"=w408:dbl[], "Polynomial Coefficients"=w450:dbl[])  [unwired: 7 in, 2 out]
        n161 = Array Max & Min(array=w416) -> (max value=w455:dbl, min value=w454:dbl)  [unwired: 2 out]
        n162 = Subtract(x=w408, y=w432) -> (x-y=w431:dbl[])
        n163 = for {
          N: w436 -> [_]
          shift-right: [w460] -> _
          shift-left: w420 -> [w461]
          tunnel: [w460] -> w440 mode=indexing
          tunnel: w419 -> [w459]
          n164 = Add(x=w461, y=w459) -> (x+y=w460:dbl)
        }
        n165 = Subtract(x=w455, y=w454) -> (x-y=w453:dbl)
        n166 = Index Array(array=w450) -> (element #1=w447:dbl, element #2=w448:dbl, element #3=w449:dbl)  [unwired: 3 in]
        n167 = Insert Into Array(array="Calibration Table", index (col)=3 ("disabled index (col)"), new element=w431) -> (w429:dbl[][])  [unwired: 1 in]
        n168 = Divide(x=w453, y=w452) -> (x/y=w451:dbl)
        n169 = Reverse 1D Array(array=w450) -> (reversed array=w410:dbl[])
        n170 = for {
          N: w452 -> [_]
          tunnel: w454 -> [w470]
          tunnel: w451 -> [w473]
          tunnel: w449 -> [w468]
          tunnel: w448 -> [w467]
          tunnel: w447 -> [w464]
          tunnel: [w463] -> w412 mode=indexing
          tunnel: [w462] -> w413 mode=indexing
          i -> [w472]
          n171 = Multiply(x=w473, y=w472) -> (x*y=w471:dbl)
          n172 = Add(x=w470, y=w471) -> (x+y=w462:dbl)
          n173 = Square(x=w462) -> (x^2=w469:dbl)
          n174 = Multiply(x=w468, y=w469) -> (x*y=w465:dbl)
          n175 = Multiply(x=w467, y=w462) -> (x*y=w466:dbl)
          n176 = Compound Arithmetic op=ADD(w464, w466, w465) -> (w463:dbl)
        }
        n177 = local write "Calibration Coefficients"(w410) -> ()
        n178 = Index Array(array=w410) -> (element #1=w441:dbl, element #2=w442:dbl, element #3=w443:dbl)  [unwired: 3 in]
        n179 = Compound Arithmetic op=MULTIPLY(w440, w440, w441) -> (w445:dbl[])
        n180 = Compound Arithmetic op=MULTIPLY(w442, w440) -> (w444:dbl[])
        n181 = Compound Arithmetic op=ADD(w445, w444, w443) -> (w422:dbl[])
        n182 = local write "Tab Control"(T2."Results" ("Tab Control")) -> ()
        n183 = Array To Spreadsheet String(delimiter (Tab)=w424, array=w422, 3:"%f" ("format string")) -> (spreadsheet string=w425:string)
        n184 = Bundle("Calibration Table"=w416, "Calibration Table"=w409) -> (w415:T12)  [unwired: 1 in]
        n185 = Bundle(w413, w412) -> (w414:cluster{dbl[], dbl[]})  [unwired: 1 in]
        n186 = Build Array(w415, w414) -> (→"M/z curve fitting":T13)
        n187 = call <vilib>:"Goodness of Fit.vi"("Best Fit"=w408, "Y"=w409) -> ("R-square"=→"R^2":dbl)  [unwired: 6 in, 3 out]
        n188 = Concatenate Strings("m/z" ("string"), w424, w425) -> (w426:string)
        n189 = Bundle By Name(cluster=w438, "m/z"=w422, "Peaks Table"=w429, "Spectrum.Calibr."=w410) -> (w446:T7)
        n190 = invoke class="App" method="Clipboard.Write"("Param 0"=w426) -> ()  [unwired: 3 in, 4 out]
      }
      event "Apply": Value Change {
        w484 = "\n"
        n191 = event-data() -> ()  [unwired: 1 in, 1 out]
        n192 = Unbundle By Name(w480) -> ("BinnedSpec.Intensity"=w489:dbl[], "Spectrum.TrigDelay"=w475:dbl, "Spectrum.SampleRate"=w476:dbl)
        n193 = Divide(x=1000000.0, y=w476) -> (x/y=w478:dbl)
        n194 = Array Size(array=w489) -> (size(s)=w488:i32)
        n195 = Multiply(x=w475, y=w478) -> (x*y=w479:dbl)
        n196 = for {
          N: w488 -> [_]
          shift-right: [w498] -> _
          shift-left: w479 -> [w499]
          tunnel: [w498] -> w491 mode=indexing
          tunnel: w478 -> [w497]
          n197 = Add(x=w499, y=w497) -> (x+y=w498:dbl)
        }
        n198 = Index Array(array="Calibration Coefficients") -> (element #1=w492:dbl, element #2=w493:dbl, element #3=w494:dbl)  [unwired: 3 in]
        n199 = Compound Arithmetic op=MULTIPLY(w491, w491, w492) -> (w496:dbl[])
        n200 = Compound Arithmetic op=MULTIPLY(w493, w491) -> (w495:dbl[])
        n201 = Compound Arithmetic op=ADD(w496, w495, w494) -> (w482:dbl[])
        n202 = Array To Spreadsheet String(delimiter (Tab)=w484, array=w482, 3:"%f" ("format string")) -> (spreadsheet string=w485:string)
        n203 = Concatenate Strings("m/z" ("string"), w484, w485) -> (w486:string)
        n204 = Bundle By Name(cluster=w480, "m/z"=w482, "Spectrum.Calibr."="Calibration Coefficients") -> (w481:T7)
        n205 = invoke class="App" method="Clipboard.Write"("Param 0"=w486) -> ()  [unwired: 3 in, 4 out]
      }
      event "Export_GraphData": Value Change {
        w503 = "\t"
        n206 = event-data() -> ()  [unwired: 1 in, 1 out]
        n207 = control-ref of="Spectrum"() -> (w516:refnum<vi>)
        n208 = property class="XYGraph (strict)"(reference=w516) -> ("Value"=w515:cluster{dbl[], "Amplitudes":dbl[]}[])  [unwired: 1 in, 2 out]
        n209 = Index Array(array=w515) -> (element=w514:cluster{dbl[], "Amplitudes":dbl[]})  [unwired: 1 in]
        n210 = Unbundle(w514) -> (w511:dbl[], "Amplitudes"=w513:dbl[])
        n211 = Array Size(array=w511) -> (size(s)=w510:i32)
        n212 = Build Array(w511, w513) -> (w512:dbl[][])
        n213 = Transpose 2D Array(2D array=w512) -> (transposed array=w508:dbl[][])
        n214 = Subtract(x=w510, y=2) -> (x-y=w506:i32)
        n215 = Array Subset(array=w508, index (row)=1 ("index"), length (row)=w506) -> (w505:dbl[][])  [unwired: 2 in]
        n216 = Unbundle By Name(w501) -> ("Filename"=w500:string)
        n217 = Array To Spreadsheet String(delimiter (Tab)=w503, array=w505, 3:"%_6g" ("format string")) -> (spreadsheet string=w518:string)
        n218 = Concatenate Strings("m/z" ("string"), w503, w500, "\r", w518) -> (w519:string)
        n219 = invoke class="App" method="Clipboard.Write"("Param 0"=w519) -> ()  [unwired: 3 in, 4 out]
      }
      event "ApplyToFile": Value Change {
        n220 = event-data() -> ()  [unwired: 1 in, 1 out]
        n221 = Unbundle By Name(w532) -> ("InitialCali."=w530:dbl[], "Spectrum"=w531:T5)
        n222 = control-ref of="Path"() -> (w529:refnum<vi>)
        n223 = property class="Path"(reference=w529) -> ("Value"=w524:path)  [unwired: 1 in, 2 out]
        n224 = Path To String(path=w524) -> (string=w527:string)
        n225 = Concatenate Strings(w527, ".bak" ("string")) -> (w526:string)
        n226 = String To Path(string=w526) -> (path=w525:path)
        n227 = Move(source path=w524, 9:TRUE ("overwrite (F)"), 10:w525) -> (error out=w522:errorcluster)  [unwired: 2 in, 2 out]
        n228 = call "WriteTextFile.vi"("overwrite? (F)"=TRUE ("Overwrite?"), "InitialCali."=w530, "error in (no error)"=w522, "Signal Segment"=w531, "Filename"=w524) -> ()  [unwired: 6 in, 1 out]
      }
      event "ApplyToMainProgram": Value Change {
        n229 = event-data() -> ()  [unwired: 1 in, 1 out]
        n230 = Unbundle By Name(w535) -> ("Spectrum.Calibr."=w534:dbl[])
        n231 = property class="Arr (strict)"(reference=w533, "Val(Sgnl)"=w534) -> ()  [unwired: 1 in, 2 out]
      }
      event "mzML Export": Value Change {
        n232 = event-data() -> ()  [unwired: 1 in, 1 out]
        n233 = Unbundle By Name(w545) -> ("Spectrum"=w543:T5)  [unwired: 1 out]
        n234 = control-ref of="Path"() -> (w544:refnum<vi>)
        n235 = property class="Path"(reference=w544) -> ("Value"=w542:path)  [unwired: 1 in, 2 out]
        n236 = Strip Path(path=w542) -> (stripped path=w541:path, name=w540:string)
        n237 = xnode "Match Regular Expression"("input string"=w540, "regular expression"="(.[0-9a-zA-Z~]+$)") -> ("before match"=w539:string, "error out"=w536:errorcluster)  [unwired: 4 in, 4 out]
        n238 = Build Path(base path=w541, name or relative path=w539) -> (appended path=w537:path)
        n239 = call "Write_mzMLFile.vi"("error in (no error)"=w536, "Signal Segment"=w543, "Filename"=w537) -> ()  [unwired: 8 in, 1 out]
      }
      event "Search": Value Change {
        n240 = event-data() -> ()  [unwired: 1 in, 1 out]
        n241 = call <vilib>:"Set Busy.vi"() -> ("error out"=w659:errorcluster)  [unwired: 10 in, 1 out]
        n242 = flat-sequence {
          tunnel: w664 -> [w678]
          tunnel: [w677] -> w662
          tunnel: [w665] -> w660
          tunnel: w659 -> [w665]
          frame #0 {
            n243 = Unbundle By Name(w678) -> ("BinnedSpec.m/z"=w676:dbl[], "BinnedSpec.Intensity"=w675:dbl[])
            n244 = call <vilib>:"Peak Detector.vi"("peaks/valleys"=enum32{"Peaks", "Valleys"}."Peaks", "width"="width", "threshold"="threshold", "X"=w675) -> ("Amplitudes"=w668:dbl[], "Locations"=w679:dbl[], "# found"=→"# found":i32)  [unwired: 3 in, 2 out]
            n245 = control-ref of="Multicolumn Listbox"() -> (w670:refnum<vi>)
            n246 = for {
              tunnel: w676 -> [w689]
              tunnel: w679 -> [w688] mode=indexing
              tunnel: [w687] -> w669 mode=indexing
              n247 = Interpolate 1D Array(1:w688, 2:w689) -> (0:w687:dbl)
            }
            n248 = Bundle(w669, "Amplitudes"=w668) -> (w677:cluster{dbl[], "Amplitudes":dbl[]})  [unwired: 1 in]
            n249 = for {
              tunnel: w669 -> [w685] mode=indexing
              tunnel: w668 -> [w684] mode=indexing
              tunnel: [w681] -> w667 mode=indexing
              n250 = Format Value(format string="%1.2f", value (0)=w685) -> (output string=w683:string)  [unwired: 1 in]
              n251 = Format Value(format string="%1.7f", value (0)=w684) -> (output string=w682:string)  [unwired: 1 in]
              n252 = Build Array(w683, w682) -> (w681:string[])
            }
            n253 = property class="MCListbox (strict)"(reference=w670, "ItemNames"=w667, "ColHdrString"=string[] ["m/z", "Intensity"]) -> ()  [unwired: 1 in, 2 out]
          }
        }
        n254 = call <vilib>:"Unset Busy.vi"("error in (no error)"=w660) -> ()  [unwired: 10 in, 1 out]
        n255 = Bundle By Name(cluster=w664, "PeaksList"=w662) -> (w663:T7)
      }
      event "ExportPCA": Value Change {
        n256 = event-data() -> ()  [unwired: 1 in, 1 out]
        n257 = call <vilib>:"Set Busy.vi"() -> ("error out"=w691:errorcluster)  [unwired: 10 in, 1 out]
        n258 = flat-sequence {
          tunnel: w694 -> [w706]
          tunnel: [w697] -> w692
          tunnel: [w695] -> w690
          tunnel: w691 -> [w695]
          frame #0 {
            w702 = 750 ("dimension size")
            n259 = for {
              N: w702 -> [_]
              shift-right: [w708] -> _
              shift-left: 50.0 -> [w707]
              tunnel: [w707] -> w698 mode=indexing
              n260 = Increment(x=w707) -> (x+1=w708:dbl)
            }
            n261 = Initialize Array(0.0 ("element"), w702) -> (w703:dbl[])
            n262 = Unbundle By Name(w706) -> ("PeaksList.m/z"=w701:dbl[], "PeaksList.Intensity"=w700:dbl[])
            n263 = for {
              N: w702 -> [_]
              shift-right: [w728] -> w699
              shift-left: w703 -> [w729]
              tunnel: w698 -> [w727]
              tunnel: w701 -> [w726] mode=indexing
              tunnel: w700 -> [w724] mode=indexing
              shift-right: [w718] -> _
              shift-left: 0.0 -> [w725]
              shift-right: [w717] -> _
              shift-left: _ -> [w716]
              i -> [w722]
              # "tracking last 10 peaks offset"
              n264 = Equal To 0?(x=w722) -> (x = 0?=w723:bool)
              n265 = Threshold 1D Array(1:w725, 2:w726, 3:w727) -> (0:w718:dbl)
              n266 = Round To Nearest(number=w718) -> (nearest integer value=w719:dbl)
              n267 = Subtract(x=w718, y=w719) -> (x-y=w711:dbl)
              n268 = Round Toward -Infinity(1:w718) -> ()  [unwired: 1 out]
              n269 = To Long Integer(number=w719) -> (32bit integer=w713:i32)
              n270 = call <vilib>:"Mean PtByPt.vi"("x"=w711, "sample length"=10, "initialize"=w723) -> ("mean"=w717:dbl)  [unwired: 1 in, 1 out]
              n271 = Sign(1:w716) -> (0:w715:dbl)
              n272 = Sign(1:w711) -> (0:w710:dbl)
              n273 = Add(x=w713, y=w710) -> (x+y=w714:dbl)
              n274 = Equal?(x=w710, y=w715) -> ()  [unwired: 1 out]
              n275 = To Long Integer(number=w714) -> (32bit integer=w712:i32)
              n276 = Select(t=w713, s=TRUE, f=w712) -> (s? t:f=w720:i32)
              n277 = in-place {
                in-place-border: w724 -> [w730]
                n278 = in-place-array #1(w729, w720) -> ()  [unwired: 1 out]
                n279 = in-place-array #1(w730) -> (w728:dbl[])  [unwired: 1 out]
              }
            }
            n280 = Bundle(w698, w699) -> (w697:cluster{dbl[], dbl[]})  [unwired: 1 in]
          }
        }
        n281 = Bundle By Name(cluster=w694, "PCA"=w692) -> (w693:T7)
        n282 = call <vilib>:"Unset Busy.vi"("error in (no error)"=w690) -> ()  [unwired: 10 in, 1 out]
      }
      event "AddSelection": Value Change {
        n283 = event-data() -> ()  [unwired: 1 in, 1 out]
        n284 = control-ref of="Multicolumn Listbox"() -> (w735:refnum<vi>)
        n285 = property class="MCListbox (strict)"(reference=w735) -> (reference out=w734:refnum<vi>, error out=w733:errorcluster, "Value"=w731:i32[])  [unwired: 1 in]
        n286 = property class="MCListbox (strict)"(reference=w734, error in=w733) -> ("ItemNames"=w732:string[][])  [unwired: 2 out]
        n287 = for {
          tunnel: w732 -> [w738] mode=indexing
          tunnel: w731 -> [w737] mode=indexing
          n288 = Array Subset(array=w738, index=w737) -> ()  [unwired: 1 in, 1 out]
        }
      }
      event "Calibration Table": Value Change {
        n289 = event-data() -> ()  [unwired: 1 in, 1 out]
        n290 = local read "Calibration Table"() -> (w739:dbl[][])
        n291 = Bundle By Name(cluster=w741, "Peaks Table"=w739) -> (w740:T7)
      }
      event "Selected Peak list": Edit Cell? {
        n292 = event-data() -> ("String"=w744:string)  [unwired: 1 in]
        n293 = xnode "Match Regular Expression"("input string"=w744, "regular expression"="([-+]?[0-9]*\\.?[0-9]+)([eE][-+]?[0-9]+)?") -> ("whole match"=w742:string)  [unwired: 4 in, 4 out]
        n294 = event-data("String"=w742) -> ()  [unwired: 2 in, 1 out]
      }
      event "CalcPeakAreas": Value Change {
        n295 = event-data() -> ()  [unwired: 1 in, 1 out]
        n296 = control-ref of="Selected Peak list"() -> (w872:refnum<vi>)
        n297 = Unbundle By Name(w870) -> ("m/z"=w865:dbl[], "Spectrum.Spectrum"=w859:sgl[])
        n298 = property class="MCListbox (strict)"(reference=w872) -> (reference out=w871:refnum<vi>, "ItemNames"=w862:string[][])  [unwired: 1 in, 1 out]
        n299 = control-ref of="CalcPeakAreas"() -> (w858:refnum<vi>)
        n300 = Index Array(array=w862, index (col) #1=0 ("disabled index (col)"), index (col) #2=1 ("index (col)")) -> (element #1=w869:string[], element #2=w866:string[])  [unwired: 2 in]
        n301 = property class="Bool (strict)"(reference=w858, "Value"=FALSE) -> ()  [unwired: 1 in, 2 out]
        n302 = for {
          tunnel: w869 -> [w889] mode=indexing
          tunnel: w866 -> [w888] mode=indexing
          tunnel: [w881] -> w864 mode=indexing if=w882
          tunnel: [w886] -> w863 mode=indexing if=w882
          w885 = nan ("default (0 DBL)")
          n303 = Fract/Exp String To Number(string=w889, default (0 dbl)=w885) -> (number=w883:dbl)  [unwired: 2 in, 1 out]
          n304 = Fract/Exp String To Number(string=w888, default (0 dbl)=w885) -> (number=w887:dbl)  [unwired: 2 in, 1 out]
          n305 = Subtract(x=w883, y=w887) -> (x-y=w881:dbl)
          n306 = Add(x=w883, y=w887) -> (x+y=w886:dbl)
          n307 = Not A Number/Path/Refnum?(number/path/refnum=w881) -> (NaN/Path/Refnum?=w884:bool)
          n308 = Not(x=w884) -> (.not. x?=w882:bool)
        }
        n309 = call "CalcPeakArea.vi"("spectrum"=w859, "m/z in"=w865, "to"=w863, "from"=w864) -> ("Peak Area"=w860:dbl[])  [unwired: 7 in]
        n310 = for {
          tunnel: w860 -> [w874] mode=indexing
          shift-right: [w875] -> w861
          shift-left: w862 -> [w877]
          i -> [w873]
          n311 = in-place {
            in-place-border: w874 -> [w878]
            n312 = in-place-array #2(w877, w873, 2) -> ()  [unwired: 1 out]
            n313 = Format Into String(format string="%_4g", w878) -> (resulting string=w879:string)  [unwired: 2 in, 1 out]
            n314 = in-place-array #2(w879) -> (w875:string[][])  [unwired: 2 out]
          }
        }
        n315 = property class="MCListbox (strict)"(reference=w871, "ItemNames"=w861) -> ()  [unwired: 1 in, 2 out]
      }
      event "CopyPeakAreas": Value Change {
        w893 = "\n"
        n316 = event-data() -> ()  [unwired: 1 in, 1 out]
        n317 = control-ref of="Selected Peak list"() -> (w900:refnum<vi>)
        n318 = property class="MCListbox (strict)"(reference=w900) -> ("ItemNames"=w898:string[][])  [unwired: 1 in, 2 out]
        n319 = Index Array(array=w898, index (col)=2 ("disabled index (col)")) -> (element=w897:string[])  [unwired: 1 in]
        n320 = for {
          tunnel: w897 -> [w905] mode=indexing
          tunnel: [w901] -> w892 mode=indexing if=w902
          n321 = Fract/Exp String To Number(string=w905, default (0 dbl)=nan ("default (0 DBL)")) -> (number=w901:dbl)  [unwired: 2 in, 1 out]
          n322 = Not A Number/Path/Refnum?(number/path/refnum=w901) -> (NaN/Path/Refnum?=w903:bool)
          n323 = Not(x=w903) -> (.not. x?=w902:bool)
        }
        n324 = Unbundle By Name(w891) -> ("Filename"=w890:string)
        n325 = Array To Spreadsheet String(delimiter (Tab)=w893, array=w892, 3:"%_4g" ("format string")) -> (spreadsheet string=w894:string)
        n326 = Concatenate Strings(w890, w893, w894) -> (w895:string)
        n327 = invoke class="App" method="Clipboard.Write"("Param 0"=w895) -> ()  [unwired: 3 in, 4 out]
      }
      event "ExportTable": Value Change {
        n328 = event-data() -> ()  [unwired: 1 in, 1 out]
        n329 = Unbundle By Name(w913) -> ("AccumulatedPeakAreas.Labels"=w906:string[], "AccumulatedPeakAreas.Areas"=w909:dbl[][])
        n330 = disable-structure "Diagram Disable Structure" shown="Enabled" {
          disable-tunnel: w909 -> [w919 w925]
          disable-tunnel: [w918 w925] -> w908
          disable-tunnel: [w917 w924] -> w907
          disable-tunnel: w906 -> [w917 w924]
          frame Disabled {
            # "Ratio calculation"
            n331 = for {
              tunnel: w919 -> [w923] mode=indexing
              tunnel: [w920] -> w918 mode=indexing
              n332 = Index Array(array=w923, index=0) -> (element=w922:dbl)
              n333 = Divide(x=w923, y=w922) -> (x/y=w920:dbl[])
            }
          }
          frame Enabled {
            # "Direct output"
          }
        }
        n334 = Transpose 2D Array(2D array=w908) -> (transposed array=w912:dbl[][])
        n335 = Array To Spreadsheet String(array=w907, 3:"%s" ("format string")) -> (spreadsheet string=w911:string)  [unwired: 1 in]
        n336 = Array To Spreadsheet String(array=w912, 3:"%_4g" ("format string")) -> (spreadsheet string=w914:string)  [unwired: 1 in]
        n337 = Concatenate Strings(w911, w914) -> (w915:string)
        n338 = invoke class="App" method="Clipboard.Write"("Param 0"=w915) -> ()  [unwired: 3 in, 4 out]
      }
      event "Export+Proc": Value Change {
        n339 = event-data() -> ()  [unwired: 1 in, 1 out]
        n340 = Unbundle By Name(w931) -> ("AccumulatedPeakAreas.Labels"=w930:string[], "AccumulatedPeakAreas.Areas"=w926:dbl[][], "AccumulatedPeakAreas.Areas^2"=w929:dbl[][], "AccumulatedPeakAreas.n"=w928:i32[])
        n341 = disable-structure "Diagram Disable Structure" shown="Enabled" {
          disable-tunnel: w926 -> [w935 w943]
          disable-tunnel: w930 -> [w937 w944]
          disable-tunnel: w929 -> [w934 _]
          disable-tunnel: w928 -> [w933 _]
          disable-tunnel: [w936 w942] -> w927
          frame Enabled {
            # "Need to test the validaty of this part"
            # "ratio calculation"
            n342 = call "GetStatistics_Array.vi"("n"=w933, "sum_X^2"=w934, "sum_X"=w935) -> ("Table"=w932:dbl[][])  [unwired: 8 in]
            n343 = Array To Spreadsheet String(array=w932, 3:"%_4g" ("format string")) -> (spreadsheet string=w939:string)  [unwired: 1 in]
            n344 = Array To Spreadsheet String(array=w937, 3:"%s\\t" ("format string")) -> (spreadsheet string=w940:string)  [unwired: 1 in]
            n345 = Concatenate Strings(w940, w939) -> (w936:string)
          }
          frame Disabled {
            # "Direct output"
            n346 = Transpose 2D Array(2D array=w943) -> (transposed array=w947:dbl[][])
            n347 = Array To Spreadsheet String(array=w944, 3:"%s" ("format string")) -> (spreadsheet string=w948:string)  [unwired: 1 in]
            n348 = Array To Spreadsheet String(array=w947, 3:"%_4g" ("format string")) -> (spreadsheet string=w946:string)  [unwired: 1 in]
            n349 = Concatenate Strings(w948, w946) -> (w942:string)
          }
        }
        n350 = invoke class="App" method="Clipboard.Write"("Param 0"=w927) -> ()  [unwired: 3 in, 4 out]
      }
      event "Accumulate": Value Change {
        n351 = event-data() -> ()  [unwired: 1 in, 1 out]
        n352 = property class="MCListbox (strict)"(reference=w961) -> ("ItemNames"=w967:string[][])  [unwired: 1 in, 2 out]
        n353 = Unbundle By Name(w965) -> ("Filename"=w959:string, "AccumulatedPeakAreas.Labels"=w960:string[], "AccumulatedPeakAreas.Areas"=w958:dbl[][], "AccumulatedPeakAreas.Areas^2"=w957:dbl[][], "AccumulatedPeakAreas.n"=w955:i32[])
        n354 = Search 1D Array(1D array=w960, element=w959) -> (index of element=w952:i32)  [unwired: 1 in]
        n355 = Index Array(array=w967, index (col)=2 ("disabled index (col)")) -> (element=w966:string[])  [unwired: 1 in]
        n356 = for {
          tunnel: w966 -> [w1002] mode=indexing
          tunnel: [w998] -> w956 mode=indexing if=w999
          n357 = Fract/Exp String To Number(string=w1002, default (0 dbl)=nan ("default (0 DBL)")) -> (number=w998:dbl)  [unwired: 2 in, 1 out]
          n358 = Not A Number/Path/Refnum?(number/path/refnum=w998) -> (NaN/Path/Refnum?=w1000:bool)
          n359 = Not(x=w1000) -> (.not. x?=w999:bool)
        }
        n360 = case shown="0.." w952 {
          selector: w952 -> [w969 _]
          tunnel: [w985 w997] -> w963
          tunnel: w960 -> [w985 w996]
          tunnel: w959 -> [w970 w986]
          tunnel: w958 -> [w983 w995]
          tunnel: w957 -> [w974 w994]
          tunnel: w956 -> [w977 w993]
          tunnel: w955 -> [w971 w991]
          tunnel: [w984 w989] -> w950
          tunnel: [w973 w988] -> w954
          tunnel: [w972 w987] -> w953
          tunnel: [w970 w986] -> w951
          frame 0.. {
            n361 = Index Array(array=w983, index (row)=w969) -> (element=w982:dbl[])  [unwired: 1 in]
            n362 = Index Array(array=w974, index (row)=w969) -> (element=w980:dbl[])  [unwired: 1 in]
            n363 = Index Array(array=w971, index=w969) -> (element=w978:i32)
            n364 = Square(x=w977) -> (x^2=w976:dbl[])
            n365 = Add(x=w982, y=w977) -> (x+y=w981:dbl[])
            n366 = Add(x=w980, y=w976) -> (x+y=w975:dbl[])
            n367 = Increment(x=w978) -> (x+1=w979:i32)
            n368 = Replace Array Subset(array=w983, new element=w981, index (row)=w969) -> (w984:dbl[][])  [unwired: 1 in]
            n369 = Replace Array Subset(array=w974, new element=w975, index (row)=w969) -> (w973:dbl[][])  [unwired: 1 in]
            n370 = Replace Array Subset(array=w971, new element=w979, index=w969) -> (w972:i32[])
          }
          frame -1, Default {
            n371 = Square(x=w993) -> (x^2=w992:dbl[])
            n372 = Build Array (concatenate)(w996, w986) -> (w997:string[])
            n373 = Build Array (concatenate)(w995, w993) -> (w989:dbl[][])
            n374 = Build Array (concatenate)(w994, w992) -> (w988:dbl[][])
            n375 = Build Array (concatenate)(w991, 1 ("element")) -> (w987:i32[])
          }
        }
        "Accumulated Data" <- w950
        n376 = Enqueue Element(queue=w962, element=w951) -> ()  [unwired: 2 in, 3 out]
        n377 = Bundle By Name(cluster=w965, "AccumulatedPeakAreas.Labels"=w963, "AccumulatedPeakAreas.Areas"=w950, "AccumulatedPeakAreas.Areas^2"=w954, "AccumulatedPeakAreas.n"=w953) -> (w964:T7)
      }
      event "Reset": Value Change {
        n378 = event-data() -> ()  [unwired: 1 in, 1 out]
        n379 = Bundle By Name(cluster=w1006, "AccumulatedPeakAreas"=T8 {"Labels"=[], "Areas"=[], "Areas^2"=[], "n"=[]}) -> (w1005:T7)
        n380 = Unbundle By Name(w1005) -> ("AccumulatedPeakAreas.Areas"=w1004:dbl[][])
        n381 = property on="Accumulated Data" class="Arr (strict)"("Value"=w1004) -> ()  [unwired: 2 in, 2 out]
      }
    }
    n382 = Unbundle By Name(w35) -> ("Peaks Table"=w40:dbl[][], "m/z"=w38:dbl[], "Spectrum.Spectrum"=w37:sgl[], "PeaksList"=w33:cluster{"m/z":dbl[], "Intensity":dbl[]}, "PCA"=w32:cluster{"m/z":dbl[], "Intensity":dbl[]})
    n383 = control-ref of="Spectrum"() -> (w31:refnum<vi>)
    n384 = local write "Calibration Table"(w40) -> ()
    n385 = case shown="True" w36 {
      tunnel: w38 -> [_ w57]
      tunnel: w37 -> [_ w56]
      tunnel: w31 -> [_ w44]
      tunnel: w35 -> [w42 w49]
      tunnel: [w42 w48] -> w34
      tunnel: w33 -> [_ w46]
      tunnel: w32 -> [_ w45]
      frame False {
      }
      frame True {
        n386 = call <vilib>:"Set Busy.vi"("disable click? (T)"=FALSE) -> ("error out"=w52:errorcluster)  [unwired: 9 in, 1 out]
        n387 = call-poly "SpecBinning.vi"("BinType"="BinType", "BinWidth"="BinWidth", "Binning"="Binning", "error in (no error)"=w52, "Signal"=w56, "m/z Array"=w57, "GraphsRef."=w44) -> ("error out"=w51:errorcluster, "BinnedSpectrum"=w43:cluster{"m/z Array":dbl[], "Signal":dbl[]})  [unwired: 3 in]
        n388 = call <vilib>:"Unset Busy.vi"("error in (no error)"=w51) -> ()  [unwired: 10 in, 1 out]
        n389 = Build Array(w43, w46, w45) -> (w47:cluster{"m/z":dbl[], "Intensity":dbl[]}[])
        n390 = disable-structure shown="Enabled" {
          disable-tunnel: w44 -> [w60 _]
          disable-tunnel: w43 -> [w59 _]
          frame Enabled {
            n391 = call-poly "FindMassResolution.vi"("EnableResDisplay"="Resolution", "BinnedSpectrum"=w59, "GraphRef."=w60) -> ()  [unwired: 7 in, 2 out]
          }
          frame Disabled {
          }
        }
        n392 = property class="XYGraph (strict)"(reference=w44, "Value"=w47) -> ()  [unwired: 1 in, 2 out]
        n393 = Bundle By Name(cluster=w49, "BinnedSpec"=w43) -> (w48:T7)
      }
    }
  }
  "Referance Mass" <- string[][] [["Compound", "", "m/z", ""], ["Sexithiophene", "6T", "493.9420", "s"], ["", "4T", "329.9665", "s"], ["", "5T-2H", "407.9230", ""], ["", "8T", "657.9174", "w"], ["C60", "M+", "720.0000", ""], ["NPM", "M+", "297.0890", "s"], ["CHCA", "M+", "189.04", "s"], ["DHB", "M+", "154.03", "s"]] ("Referance Mass")
